vi "Open.vi"(8 "error in (no error)":errorcluster, 10 "timeout (10sec)":u32=10000, 11 "VISA resource name":refnum<visa-resource-name>) -> (0 "error out":errorcluster, 3 "VISA resource name out":refnum<visa-resource-name>)   [LabVIEW 2026]
uses:
  <vilib>/Instr/_visa.llb/VISA Configure Serial Port (Instr).vi
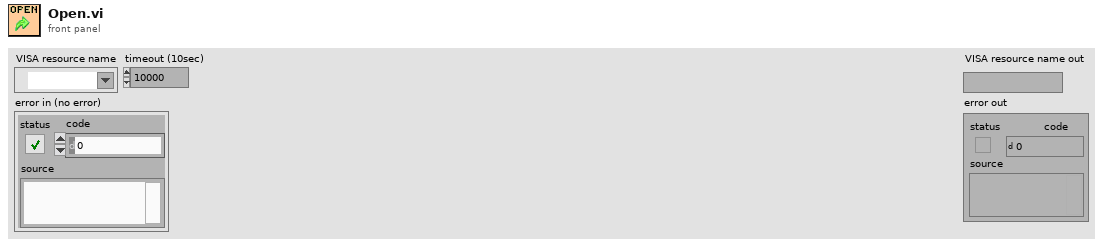
[diagram p1: front panel]
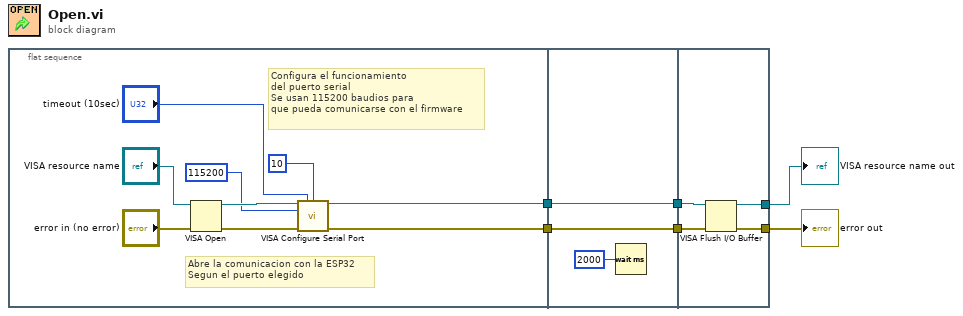
[diagram p0: block diagram]
diagram:
  n1 = flat-sequence {
    tunnel: [w12] -> w4
    tunnel: [w11] -> w3
    tunnel: w4 -> [w18]
    tunnel: w3 -> [w17]
    tunnel: [w18] -> w2
    tunnel: [w17] -> w1
    tunnel: [w20] -> w5
    tunnel: [w19] -> w6
    tunnel: w2 -> [w22]
    tunnel: w1 -> [w21]
    frame #0 {
      # "Configura el funcionamiento \ndel puerto serial \nSe usan 115200 baudios para \nque pueda comunicarse con el firmware"
      # "Abre la comunicacion con la ESP32\nSegun el puerto elegido"
      n2 = VISA Open(error in (no error)="error in (no error)", VISA resource name="VISA resource name") -> (VISA resource name=w15:refnum<visa-resource-name>, error out=w14:errorcluster)  [unwired: 3 in]
      n3 = call-poly "VISA Configure Serial Port"("VISA resource name"=w15, "timeout (10sec)"="timeout (10sec)", "termination char\n(0xA = '\\n' = LF)"=u8 10 ("termination char\n(0xA = '\\n' = LF)"), "baud rate (9600)"=u32 115200, "error in (no error)"=w14) -> ("VISA resource name out"=w12:refnum<visa-resource-name>, "error out"=w11:errorcluster)  [unwired: 9 in]
    }
    frame #1 {
      n4 = Wait (ms)(milliseconds to wait=u32 2000) -> ()  [unwired: 1 out]
    }
    frame #2 {
      n5 = VISA Flush I/O Buffer(VISA resource name=w22, error in (no error)=w21) -> (VISA resource name out=w19:refnum<visa-resource-name>, error out=w20:errorcluster)  [unwired: 1 in]
    }
  }
  "VISA resource name out" <- w6
  "error out" <- w5
